vi "RT_ShVariables.vi"() -> ()   [LabVIEW 2025]
panel:
  out "error out":errorcluster
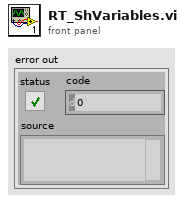
[diagram p1: front panel]
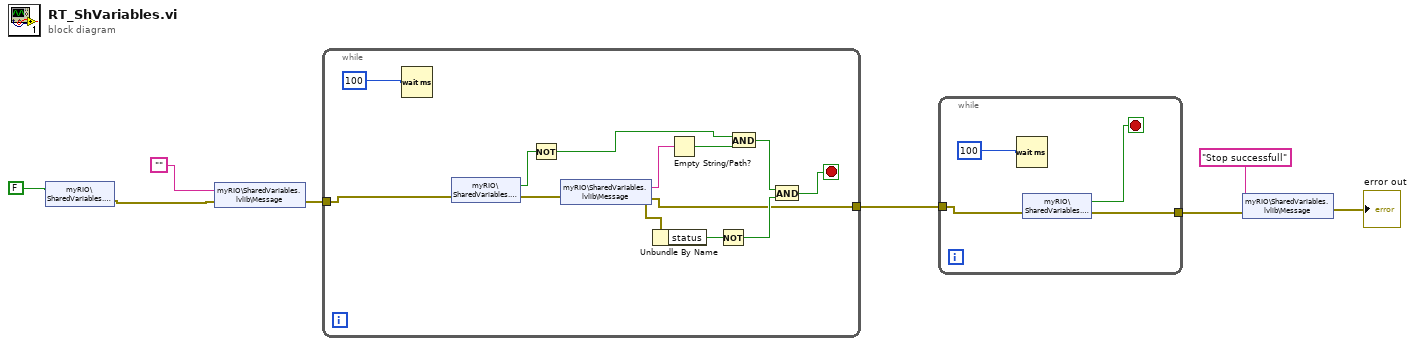
[diagram p0: block diagram]
diagram:
  n1 = shared-variable "myRIO\\SharedVariables.lvlib\\Stop"(FALSE ("Stop")) -> (error out=w7:errorcluster)  [unwired: 1 in]
  n2 = shared-variable "myRIO\\SharedVariables.lvlib\\Message"("", error in=w7) -> (error out=w6:errorcluster)
  n3 = while {
    tunnel: w6 -> [w20]
    tunnel: [w9] -> w4
    stop <- w11 stop-if-true
    n4 = Wait (ms)(milliseconds to wait=u32 100) -> ()  [unwired: 1 out]
    n5 = shared-variable "myRIO\\SharedVariables.lvlib\\Stop"(error in=w20) -> (w18:bool, error out=w19:errorcluster)
    n6 = Not(x=w18) -> (.not. x?=w14:bool)
    n7 = shared-variable "myRIO\\SharedVariables.lvlib\\Message"(error in=w19) -> (w17:string, error out=w9:errorcluster)
    n8 = Unbundle By Name(w9) -> ("status"=w16:bool)
    n9 = Empty String/Path?(string/path=w17) -> (empty?=w15:bool)
    n10 = Not(x=w16) -> (.not. x?=w12:bool)
    n11 = And(x=w14, y=w15) -> (x .and. y?=w13:bool)
    n12 = And(x=w13, y=w12) -> (x .and. y?=w11:bool)
  }
  n13 = while {
    tunnel: w4 -> [w24]
    tunnel: [w21] -> w3
    stop <- w23 stop-if-true
    n14 = Wait (ms)(milliseconds to wait=u32 100) -> ()  [unwired: 1 out]
    n15 = shared-variable "myRIO\\SharedVariables.lvlib\\Stop"(error in=w24) -> (w23:bool, error out=w21:errorcluster)
  }
  n16 = shared-variable "myRIO\\SharedVariables.lvlib\\Message"("Stop successfull" ("Message"), error in=w3) -> (error out=→"error out":errorcluster)
